vi "Acquisition_Gentec.vi"(0 "DATA Folder Path":string="D:\\MDSPLUS_PHASMA\\RAWDATA\\", 1 "time stamp":timestamp, 3 "Shot Number":i32, 4 "MDSPLUS-Store?":bool=TRUE, 5 "File-Store?":bool=TRUE, 6 "VISA_Gentec (COM)":string="ASRL30::INSTR") -> (2 "Energy (J)":dbl)   [LabVIEW 2019]
panel:
  out "Read Buffer":string
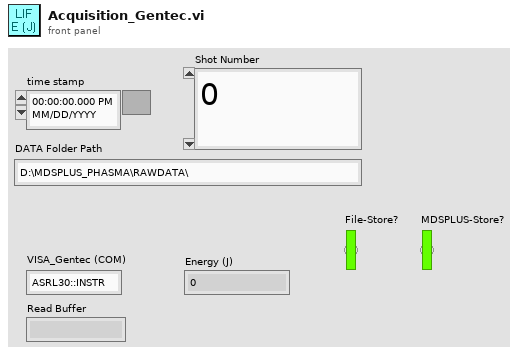
[diagram p1: front panel]
types:
  T1 = enum16{"open", "replace", "create", "open or create", "replace or create", "replace or create with confirmation"}
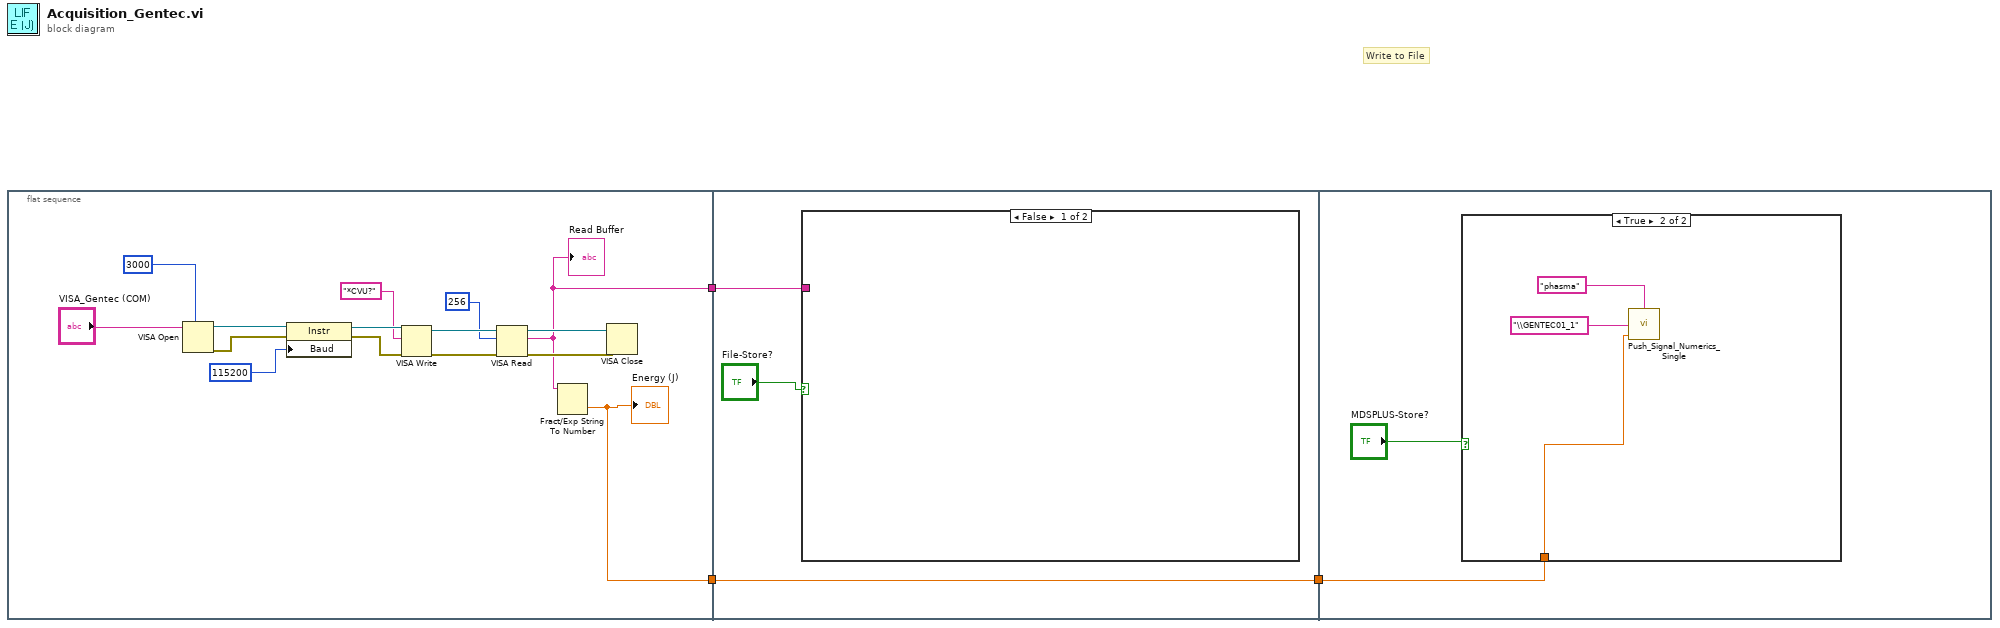
[diagram p0: block diagram]
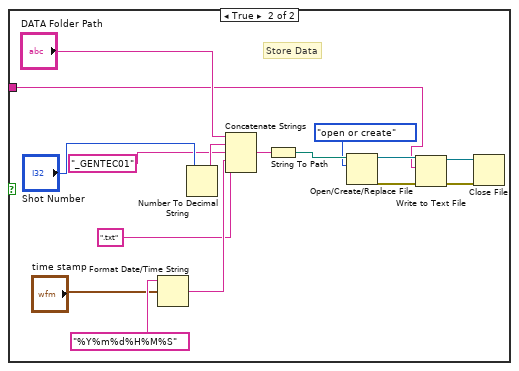
[diagram p2: hidden frame]
diagram:
  # "Write to File"
  n1 = flat-sequence {
    tunnel: [w5] -> w3
    tunnel: [w4] -> w2
    tunnel: w3 -> [w19]
    tunnel: w2 -> [w20]
    tunnel: [w19] -> w1
    tunnel: w1 -> [w38]
    frame #0 {
      n2 = VISA Open(timeout (0)=u32 3000 ("VISA Open timeout (0)"), VISA resource name="VISA_Gentec (COM)") -> (VISA resource name=w16:refnum<visa-resource-name>, error out=w15:errorcluster)  [unwired: 3 in]
      n3 = property class="Instr"(reference=w16, error in=w15, "Baud"=u32 115200 ("Serial Settings:Baud Rate")) -> (reference out=w13:refnum<visa-resource-name>, error out=w10:errorcluster)
      n4 = VISA Write(VISA resource name=w13, write buffer="*CVU?", error in (no error)=w10) -> (VISA resource name out=w12:refnum<visa-resource-name>, error out=w9:errorcluster)  [unwired: 1 out]
      n5 = VISA Read(VISA resource name=w12, byte count=u32 256, error in (no error)=w9) -> (VISA resource name out=w7:refnum<visa-resource-name>, read buffer=w4:string, error out=w6:errorcluster)  [unwired: 1 out]
      "Read Buffer" <- w4
      n6 = Fract/Exp String To Number(string=w4) -> (number=w5:dbl)  [unwired: 3 in, 1 out]
      "Energy (J)" <- w5
      n7 = VISA Close(VISA resource name=w7, error in (no error)=w6) -> ()  [unwired: 1 out]
    }
    frame #1 {
      n8 = case shown="False" "File-Store?" {
        tunnel: w20 -> [_ w22]
        frame False {
        }
        frame True {
          # "Store Data"
          n9 = Format Date/Time String(time format string (%c)="%Y%m%d%H%M%S", seconds (now)="time stamp") -> (date/time string=w33:string)  [unwired: 1 in]
          n10 = Number To Decimal String(number="Shot Number") -> (decimal integer string=w36:string)  [unwired: 1 in]
          n11 = Concatenate Strings("DATA Folder Path", w36, "_GENTEC01", w33, ".txt") -> (w37:string)
          n12 = String To Path(string=w37) -> (path=w35:path)
          n13 = Open/Create/Replace File(file path (use dialog)=w35, operation (0:open)=T1."open or create") -> (refnum out=w26:refnum<file>, error out=w25:errorcluster)  [unwired: 4 in, 1 out]
          n14 = Write to Text File(file (use dialog)=w26, text=w22, error in=w25) -> (refnum out=w23:refnum<file>, error out=w24:errorcluster)  [unwired: 1 in, 1 out]
          n15 = Close File(refnum=w23, error in=w24) -> ()  [unwired: 2 out]
        }
      }
    }
    frame #2 {
      n16 = case shown="True" "MDSPLUS-Store?" {
        tunnel: w38 -> [_ w40]
        frame False {
        }
        frame True {
          n17 = call "Push_Signal_Numerics_Single.vi"("Value In"=w40, "Path"="\\GENTEC01_1" ("Node Tag"), "Tree Name"="phasma") -> ()
        }
      }
    }
  }
